vi "Get Bundler.vi"(8 "error in (no error)":errorcluster, 10 "label":string, 11 "owner vi in":refnum<vi>) -> (0 "error out":errorcluster, 1 "found?":bool, 2 "bundler ref":refnum<vi>, 3 "owner vi out":refnum<vi>)   [LabVIEW 2019, in "gRPC Template Creation Utility.lvlib"]
uses:
  gRPC Template Creation Utility.lvlib
  <vilib>/Utility/traverseref.llb/TRef TravTarget.ctl
  <vilib>/Utility/traverseref.llb/VI Scripting - Traverse.lvlib
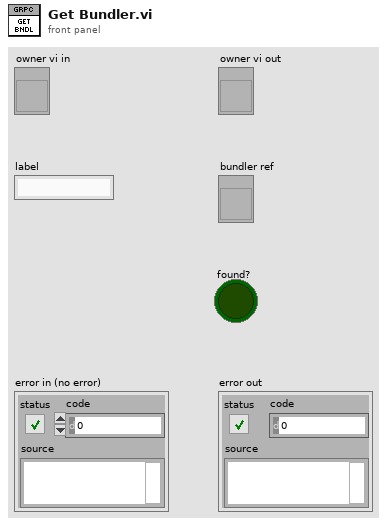
[diagram p1: front panel]
types:
  T1 = typedef "TRef TravTarget.ctl" = enum16{"FP", "BD", "Other"}
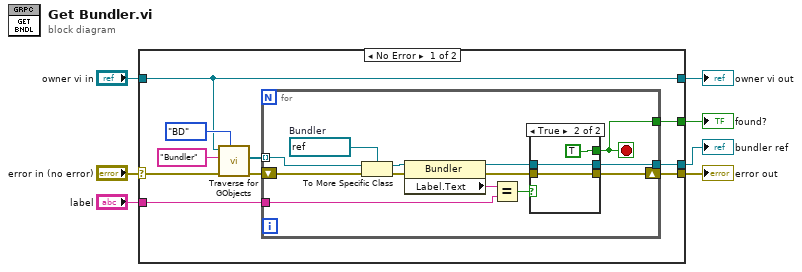
[diagram p0: block diagram]
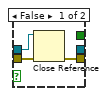
[diagram p2: hidden frame]
diagram:
  n1 = case shown="No Error" "error in (no error)" {
    selector: "error in (no error)" -> [w11 w37]
    tunnel: "label" -> [w17 _]
    tunnel: "owner vi in" -> [w10 w38]
    tunnel: [w8 w37] -> w5
    tunnel: [w12 _] -> w1
    tunnel: [w10 w38] -> w3
    tunnel: [w9 _] -> w2
    frame No Error {
      n2 = call <vilib>:"Traverse for GObjects.vi"("Traverse Target"=TRef_TravTarget."BD", "error in (no error)"=w11, "Class Name"="Bundler", "VI Refnum"=w10) -> ("error out"=w13:errorcluster, "References"=w16:refnum<vi>[])  [unwired: 4 in, 2 out]
      n3 = for {
        tunnel: w16 -> [w30] mode=indexing
        tunnel: w17 -> [w25]
        tunnel: [w22] -> w12
        tunnel: [w20] -> w9
        shift-right: [w18] -> w8
        shift-left: w13 -> [w28]
        stop <- w20 stop-if-true
        w29 = refnum<vi> refnum  # Bundler
        n4 = To More Specific Class(target class=w29, reference=w30, error in=w28) -> (specific class reference=w27:refnum<vi>, error out=w19:errorcluster)
        n5 = property class="Bundler"(reference=w27, error in=w19) -> (reference out=w23:refnum<vi>, error out=w21:errorcluster, "Label.Text"=w26:string)
        n6 = Equal?(x=w26, y=w25) -> (x = y?=w24:bool)
        n7 = case shown="True" w24 {
          tunnel: w23 -> [w33 w36]
          tunnel: [_ w36] -> w22
          tunnel: [_ TRUE] -> w20
          tunnel: w21 -> [w32 w34]
          tunnel: [w31 w34] -> w18
          frame False {
            n8 = Close Reference(reference=w33, error in (no error)=w32) -> (error out=w31:errorcluster)
          }
          frame True {
          }
        }
      }
    }
    frame Error {
    }
  }
  "error out" <- w5
  "owner vi out" <- w3
  "found?" <- w2
  "bundler ref" <- w1
